vi "RT_Pressure_PID_Loop.vi"(8 "error in (no error)":errorcluster={"status"=FALSE, "code"=0, "source"="\"\""}, 10 "PRV feedback":string, 11 "Pressure SP/PV":string) -> (0 "error out":errorcluster={"status"=FALSE, "code"=0, "source"="\"\""}, 2 "status ok":bool, 3 "AO demand and status":string)   [LabVIEW 2026]
doc: "INTENT: Regulate pressure using PRV AO. LOGIC: Apply mode transition, saturate/anti-windup, verify sensor quality and convert output to analog scale."
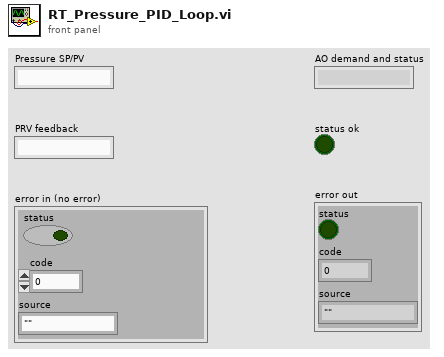
[diagram p1: front panel]
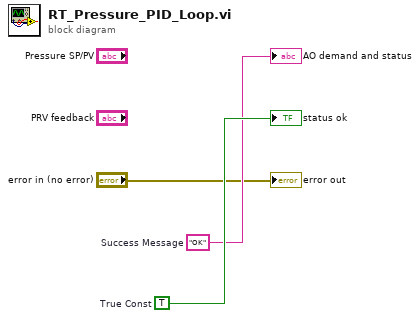
[diagram p0: block diagram]
diagram:
  w3 = TRUE  # True Const
  w2 = "OK"  # Success Message
  "AO demand and status" <- w2
  "status ok" <- w3
  "error out" <- "error in (no error)"
